vi "C_HDLC_Decode.vi"(8 "error in (no error)":errorcluster, 10 "state in":T1, 11 "bytes in":T2 format="%.0x") -> (0 "error out":errorcluster, 1 "crc errors":u32, 2 "state out":T1, 3 "payloads":T3[](array[typedef]))   [LabVIEW 2021, in "CANsub_C.lvlib"]
doc: "Feeds received bytes into the HDLC decoder and returns every complete payload with a valid CRC. Bytes of an incomplete frame stay in the state for the next call. crc errors is cumulative. Allocates on every call: tests only."
uses:
  CANsub_C.lvlib
  codec_vis/CANsub_Codec.lvlib
  common/Typedefs/Bytes.ctl
  common/CANsub_Common.lvlib
  common/Typedefs/Payload.ctl
  C_State.ctl
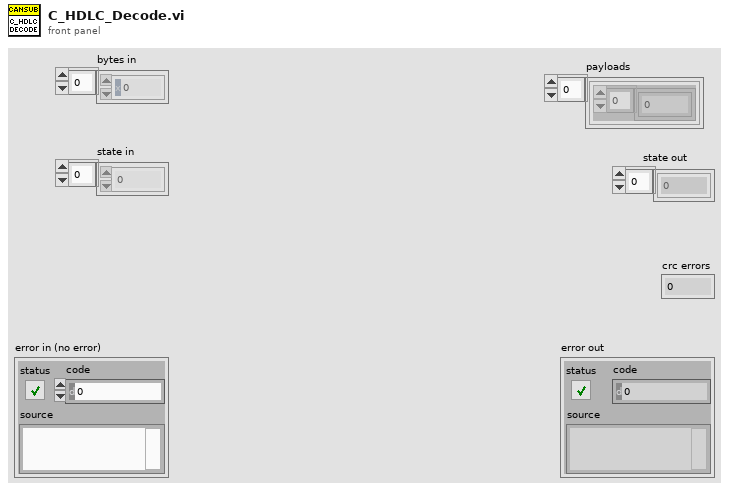
[diagram p1: front panel]
types:
  T1 = typedef "CANsub_C.lvlib/C_State.ctl" = u8[]
  T2 = typedef "CANsub_Common.lvlib/Bytes.ctl" = u8[]
  T3 = typedef "CANsub_Common.lvlib/Payload.ctl" = cluster{"payload":T2}
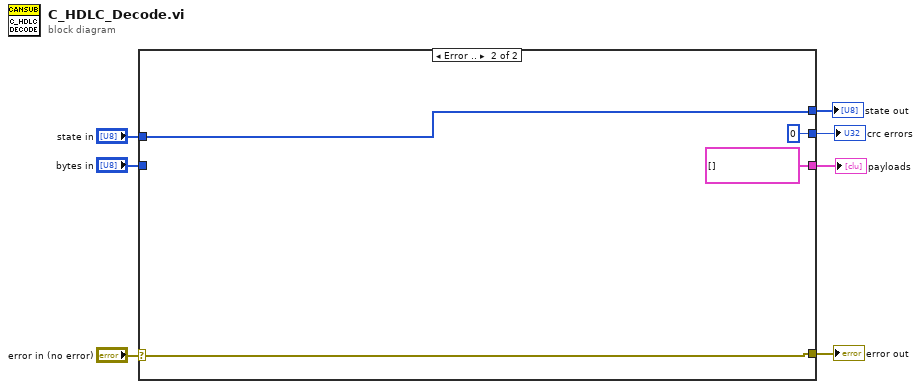
[diagram p0: block diagram]
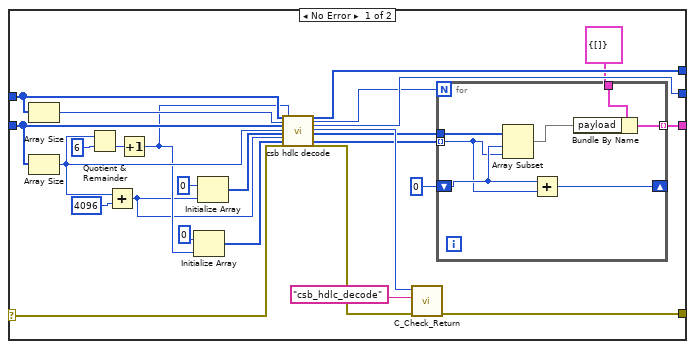
[diagram p2: hidden frame]
diagram:
  n1 = case shown="Error .." "error in (no error)" {
    selector: "error in (no error)" -> [w19 w44]
    tunnel: [w17 w44] -> w6
    tunnel: "bytes in" -> [w26 _]
    tunnel: "state in" -> [w25 w41]
    tunnel: [w13 u32 0 ("crc_errors")] -> w3
    tunnel: [w12 w41] -> w2
    tunnel: [w9 T3[] []] -> w1
    frame No Error {
      n2 = Array Size(array=w25) -> (size(s)=w24:i32)
      n3 = Array Size(array=w26) -> (size(s)=w23:i32)
      n4 = Quotient & Remainder(x=w23, y=6) -> (floor(x/y)=w29:i32)  [unwired: 1 out]
      n5 = Add(x=w23, y=4096) -> (x+y=w20:i32)
      n6 = Increment(x=w29) -> (x+1=w21:i32)
      n7 = Initialize Array(0, w21) -> (w22:i32[])
      n8 = Initialize Array(u8 0, w20) -> (w28:u8[])
      n9 = call "csb hdlc decode.vi"("state"=w25, "state_size"=w24, "in"=w26, "in_len"=w23, "out"=w28, "out_cap"=w20, "lens"=w22, "error in (no error)"=w19, "lens_cap"=w21) -> ("state out"=w12:u8[], "n_payloads"=w8:i32, "crc_errors"=w13:u32, "function return"=w27:i32, "out out"=w15:u8[], "lens out"=w14:i32[], "error out"=w18:errorcluster)  [unwired: 12 in]
      n10 = call "C_Check_Return.vi"("error in (no error)"=w18, "function name"="csb_hdlc_decode", "function return"=w27) -> ("error out"=w17:errorcluster)  [unwired: 6 in, 2 out]
      n11 = for {
        N: w8 -> [_]
        tunnel: w15 -> [w40]
        tunnel: w14 -> [w36] mode=indexing
        tunnel: T3 {"payload"=[]} ("Payload") -> [w39]
        shift-right: [w35] -> _
        shift-left: 0 -> [w37]
        tunnel: [w34] -> w9 mode=indexing
        n12 = Array Subset(array=w40, index=w37, length=w36) -> (w38:u8[])
        n13 = Add(x=w37, y=w36) -> (x+y=w35:i32)
        n14 = Bundle By Name(cluster=w39, "payload"=w38) -> (w34:T3)
      }
    }
    frame Error {
    }
  }
  "state out" <- w2
  "error out" <- w6
  "payloads" <- w1
  "crc errors" <- w3
